vi "Element Type.vi"(11 "DblNumericStatusIndicator in":refnum<class "DblStatusIndicator.lvclass">) -> (2 "Indicator Type":string)   [LabVIEW 2020, in "VolatusGUIElements.lvlib" / "DblStatusIndicator.lvclass"]
uses:
  DblStatusIndicator.lvclass
  DblStatusIndicator.lvclass/DblStatusIndicator.ctl
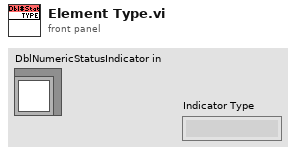
[diagram p1: front panel]
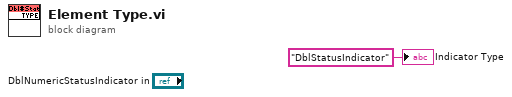
[diagram p0: block diagram]
diagram:
  "Indicator Type" <- "DblStatusIndicator" ("Indicator Type")
